vi "Check Change Result.vi"(8 "error in (no error)":errorcluster, 9 "Old Val":T4, 10 "New Val":T4, 11 "GroupLoggingControl in":refnum<class "GroupLoggingControl.lvclass">) -> (0 "error out":errorcluster, 1 "Node (Empty = All)":string, 2 "Log Group":T1, 3 "GroupLoggingControl out":refnum<class "GroupLoggingControl.lvclass">)   [LabVIEW 2020, in "VolatusGUIElements.lvlib" / "GroupLoggingControl.lvclass"]
uses:
  GroupLoggingControl.lvclass
  Log Group.ctl
  Log Group Status.ctl
  Command Info.ctl
  GroupLoggingControl.lvclass/GroupLoggingControl.ctl
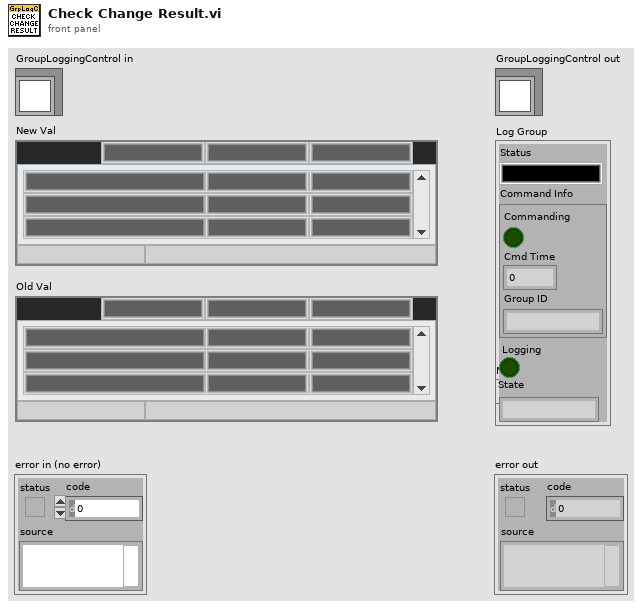
[diagram p1: front panel]
types:
  T1 = typedef "VolatusGUIElements.lvlib/GroupLoggingControl.lvclass/Log Group.ctl" = cluster{"Status":T2, "Command Info":T3, "Logging":bool, "State":string}
  T2 = typedef "VolatusGUIElements.lvlib/GroupLoggingControl.lvclass/Log Group Status.ctl" = cluster{"Group":string, "Group Color":u32, "Button":bool}
  T3 = typedef "VolatusGUIElements.lvlib/GroupLoggingControl.lvclass/Command Info.ctl" = cluster{"Commanding":bool, "Cmd Time":dbl, "Group ID":string}
  T4 = cluster{"Series":string, "Timestamp":string, "Targets":cluster{"Node":string, "Node Color":u32, "Groups":cluster{"Group":string, "Group Color":u32, "Button":bool}[]}[], "Groups":cluster{"Group":string, "Group Color":u32, "Button":bool}[]}
  T5 = cluster{"Series":bool, "Timestamp":bool, "Targets":cluster{"Node":bool, "Node Color":bool, "Groups":cluster{"Group":bool, "Group Color":bool, "Button":bool}[]}[], "Groups":cluster{"Group":bool, "Group Color":bool, "Button":bool}[]}
  T6 = typedef "VolatusGUIElements.lvlib/GroupLoggingControl.lvclass/Status.ctl" = cluster{"Groups":T1[], "Targets":T7[]}
  T7 = typedef "VolatusGUIElements.lvlib/GroupLoggingControl.lvclass/Target Info.ctl" = cluster{"Node":string, "Node Color":u32, "Groups":T1[]}
  T8 = cluster{"Node":bool, "Node Color":bool, "Groups":cluster{"Group":bool, "Group Color":bool, "Button":bool}[]}[]
  T9 = cluster{"Group":bool, "Group Color":bool, "Button":bool}[]
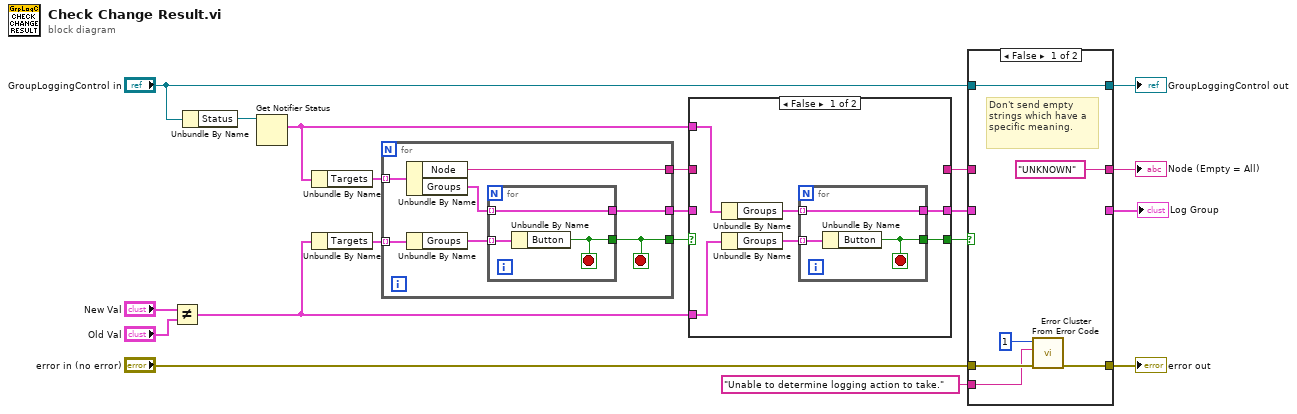
[diagram p0: block diagram]
diagram:
  n1 = Not Equal?(x="New Val", y="Old Val") -> (x != y?=w13:T5)
  n2 = Unbundle By Name("GroupLoggingControl in") -> ("Status"=w2:refnum<notifier>)
  n3 = Get Notifier Status(notifier=w2) -> (current notification=w1:T6)  [unwired: 1 in, 4 out]
  n4 = Unbundle By Name(w1) -> ("Targets"=w17:T7[])
  n5 = Unbundle By Name(w13) -> ("Targets"=w19:T8)
  n6 = for {
    tunnel: w19 -> [w27] mode=indexing
    tunnel: w17 -> [w25] mode=indexing
    tunnel: [w23] -> w14
    tunnel: [w22] -> w15
    tunnel: [w21] -> w16
    stop <- w21 stop-if-true
    n7 = Unbundle By Name(w25) -> ("Node"=w23:string, "Groups"=w24:T1[])
    n8 = Unbundle By Name(w27) -> ("Groups"=w26:T9)
    n9 = for {
      tunnel: w26 -> [w30] mode=indexing
      tunnel: w24 -> [w28] mode=indexing
      tunnel: [w28] -> w22
      tunnel: [w29] -> w21
      stop <- w29 stop-if-true
      n10 = Unbundle By Name(w30) -> ("Button"=w29:bool)
    }
  }
  n11 = case shown="False" w16 {
    selector: w16 -> [_ w40]
    tunnel: w15 -> [_ w41]
    tunnel: w14 -> [_ w42]
    tunnel: [_ w42] -> w11
    tunnel: [w32 w41] -> w10
    tunnel: w1 -> [w36 _]
    tunnel: w13 -> [w35 _]
    tunnel: [w31 w40] -> w12
    frame False {
      n12 = Unbundle By Name(w36) -> ("Groups"=w33:T1[])
      n13 = Unbundle By Name(w35) -> ("Groups"=w34:T9)
      n14 = for {
        tunnel: w34 -> [w39] mode=indexing
        tunnel: w33 -> [w37] mode=indexing
        tunnel: [w37] -> w32
        tunnel: [w38] -> w31
        stop <- w38 stop-if-true
        n15 = Unbundle By Name(w39) -> ("Button"=w38:bool)
      }
    }
    frame True {
      # "Target specific Group command"
    }
  }
  n16 = case shown="False" w12 {
    tunnel: w11 -> [_ w52]
    tunnel: w10 -> [_ w51]
    tunnel: ["UNKNOWN" ("Node") w52] -> w9
    tunnel: [_ w51] -> w3
    tunnel: "GroupLoggingControl in" -> [w48 w50]
    tunnel: [w48 w50] -> w7
    tunnel: "error in (no error)" -> [w46 w49]
    tunnel: [w45 w49] -> w5
    tunnel: "Unable to determine logging action to take." -> [w43 _]
    frame False {
      # "Don't send empty strings which have a specific meaning."
      n17 = call <vilib>:"Error Cluster From Error Code.vi"("error in (no error)"=w46, "error message (\"\")"=w43, "error code (0)"=1) -> ("error out"=w45:errorcluster)  [unwired: 6 in]
    }
    frame True {
    }
  }
  "error out" <- w5
  "GroupLoggingControl out" <- w7
  "Node (Empty = All)" <- w9
  "Log Group" <- w3
